vi "Getter Generation tester.vi"() -> ()   [LabVIEW 2020, in "Method Generation.lvlib" / "Getter Generator.lvclass"]
uses:
  Getter Generator.lvclass
  Getter Generator.lvclass/Getter Generator.ctl
panel:
  out "error out":errorcluster
  out "Attributes":map{string, refnum<vi>}(c390)
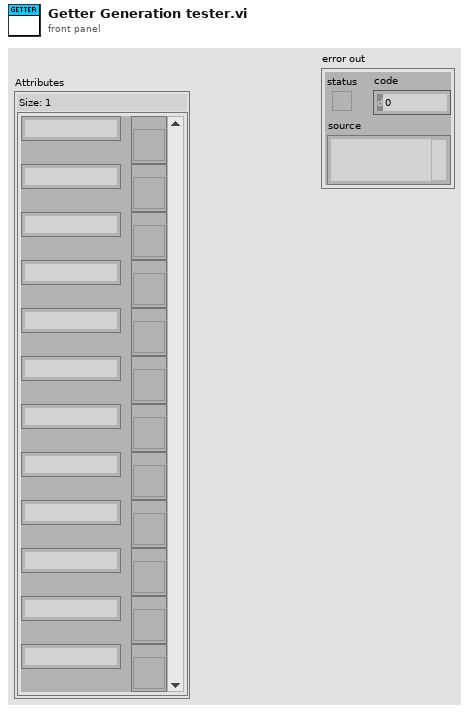
[diagram p1: front panel]
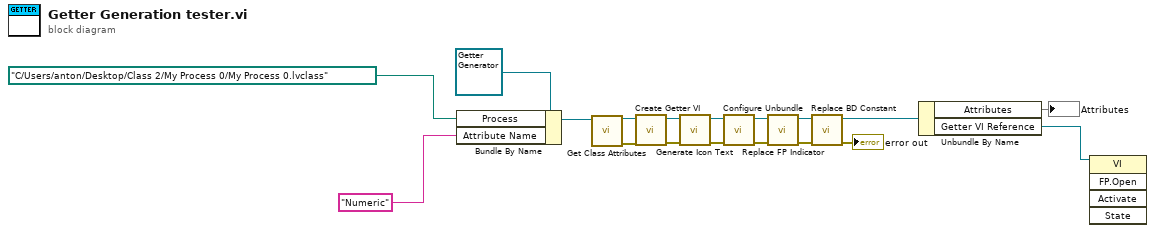
[diagram p0: block diagram]
diagram:
  n1 = Bundle By Name(cluster=refnum<class "Getter Generator.lvclass"> refnum ("New Getter Dialog In"), "Process"=path "C:/Users/anton/Desktop/Class 2/My Process 0/My Process 0.lvclass", "Attribute Name"="Numeric") -> (w17:refnum<class "Getter Generator.lvclass">)
  n2 = call "Get Class Attributes.vi"("New Getter Dialog In"=w17) -> ("error out"=w14:errorcluster, "New Getter Dialog Out"=w15:refnum<class "Getter Generator.lvclass">)  [unwired: 9 in]
  n3 = call "Create Getter VI.vi"("error in (no error)"=w14, "New Getter Dialog in"=w15) -> ("error out"=w12:errorcluster, "New Getter Dialog out"=w2:refnum<class "Getter Generator.lvclass">)  [unwired: 8 in]
  n4 = call "Generate Icon Text.vi"("error in (no error)"=w12, "Getter Generator in"=w2) -> ("error out"=w3:errorcluster, "Getter Generator out"=w1:refnum<class "Getter Generator.lvclass">)  [unwired: 8 in]
  n5 = call "Configure Unbundle.vi"("error in (no error)"=w3, "Getter Generator in"=w1) -> ("error out"=w7:errorcluster, "Getter Generator out"=w10:refnum<class "Getter Generator.lvclass">)  [unwired: 8 in]
  n6 = call "Replace FP Indicator.vi"("error in (no error)"=w7, "Getter Generator In"=w10) -> ("error out"=w6:errorcluster, "Getter Generator Out"=w9:refnum<class "Getter Generator.lvclass">)  [unwired: 8 in]
  n7 = call "Replace BD Constant.vi"("error in (no error)"=w6, "Getter Generator In"=w9) -> ("error out"=→"error out":errorcluster, "Getter Generator Out"=w8:refnum<class "Getter Generator.lvclass">)  [unwired: 8 in]
  n8 = Unbundle By Name(w8) -> ("Attributes"=→"Attributes":map{string, refnum<vi>}, "Getter VI Reference"=w11:refnum<vi>)
  n9 = invoke class="VI" method="FP.Open"(reference=w11) -> ()  [unwired: 4 in, 5 out]
